vi "Remove User from Group.vi"(5 "Save File":bool=TRUE, 6 "error in (no error)":errorcluster, 7 "Group Name":string, 8 "LoginName":string, 9 "EasyUserManager in":refnum<class "EasyUserManager.lvclass">) -> (0 "error out":errorcluster, 3 "EasyUserManager out":refnum<class "EasyUserManager.lvclass">)   [LabVIEW 2024, in "EasyUserManager.lvclass"]
doc: "Remove the user specified by <B>LoginName</B> from the group specified by <B>Group Name</B>.\n\nThis VI will not do anything if the user is not a member of the group. \n\nThe boolean input <B>Save File</B> controls whether changes are immediately saved to the users file (Default: True)."
uses:
  EasyUserManager.lvclass
  EasyUserManager.lvclass/EasyUserManager.ctl
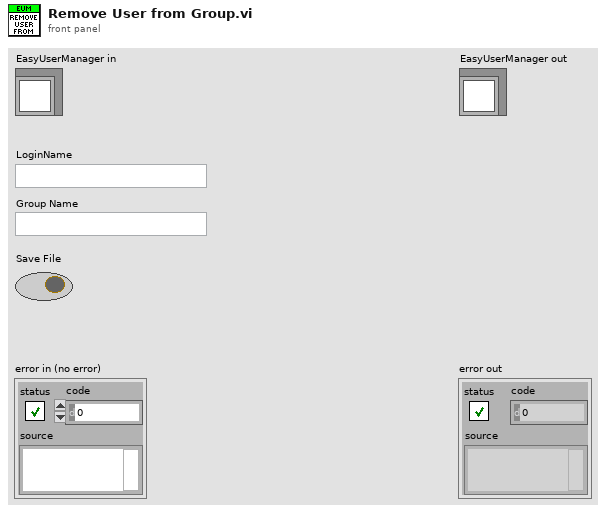
[diagram p1: front panel]
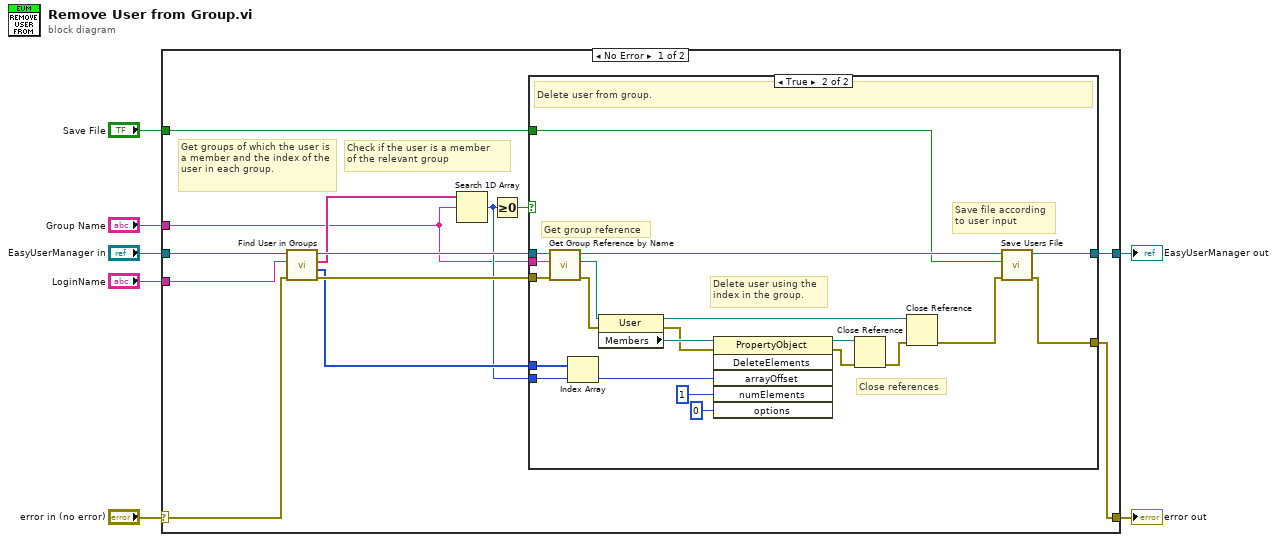
[diagram p0: block diagram]
diagram:
  n1 = case shown="No Error" "error in (no error)" {
    selector: "error in (no error)" -> [w11 w45]
    tunnel: [w19 w45] -> w6
    tunnel: [w20 w44] -> w4
    tunnel: "EasyUserManager in" -> [w17 w44]
    tunnel: "Save File" -> [w10 _]
    tunnel: "LoginName" -> [w9 _]
    tunnel: "Group Name" -> [w8 _]
    frame No Error {
      # "Check if the user is a member\nof the relevant group"
      # "Get groups of which the user is a member and the index of the user in each group."
      n2 = call "Find User in Groups.vi"("error in (no error)"=w11, "LoginName"=w9, "EasyUserManager in"=w17) -> ("error out"=w16:errorcluster, "Indexes"=w13:i32[], "Groups"=w15:string[], "EasyUserManager out"=w18:refnum<class "EasyUserManager.lvclass">)  [unwired: 1 in]
      n3 = Search 1D Array(1D array=w15, element=w8) -> (index of element=w12:i32)  [unwired: 1 in]
      n4 = Greater Or Equal To 0?(x=w12) -> (x >= 0?=w14:bool)
      n5 = case shown="True" w14 {
        tunnel: [w22 w43] -> w20
        tunnel: [w21 w42] -> w19
        tunnel: w18 -> [w22 w30]
        tunnel: w16 -> [w21 w29]
        tunnel: w8 -> [_ w27]
        tunnel: w13 -> [_ w26]
        tunnel: w12 -> [_ w25]
        tunnel: w10 -> [_ w23]
        frame False {
          # "User is not a member of the group. Do nothing."
        }
        frame True {
          # "Delete user using the \nindex in the group."
          # "Get group reference"
          # "Close references"
          # "Save file according\nto user input"
          # "Delete user from group."
          n6 = call "Get Group Reference by Name.vi"("error in (no error)"=w29, "Group Name"=w27, "EasyUserManager in"=w30) -> ("error out"=w32:errorcluster, "Group Reference"=w33:refnum<k7>, "EasyUserManager out"=w41:refnum<class "EasyUserManager.lvclass">)  [unwired: 2 in]
          n7 = Index Array(array=w26, index=w25) -> (element=w24:i32)
          n8 = property on="Property Node" class="User"(reference=w33, error in=w32) -> (reference out=w34:refnum<k7>, error out=w39:errorcluster, "Members"=w40:refnum<k7>)
          n9 = invoke on="Invoke Node" class="PropertyObject" method="DeleteElements"(reference=w40, error in=w39, "arrayOffset"=w24, "numElements"=1 ("options"), "options"=0 ("arrayOffset")) -> (reference out=w37:refnum<k7>, error out=w36:errorcluster)  [unwired: 1 in, 4 out]
          n10 = Close Reference(reference=w37, error in (no error)=w36) -> (error out=w35:errorcluster)
          n11 = Close Reference(reference=w34, error in (no error)=w35) -> (error out=w31:errorcluster)
          n12 = call "Save Users File.vi"("error in (no error)"=w31, "Save"=w23, "EasyUserManager in"=w41) -> ("error out"=w42:errorcluster, "EasyUserManager out"=w43:refnum<class "EasyUserManager.lvclass">)  [unwired: 3 in]
        }
      }
    }
    frame Error {
      # "Pass error and do nothing."
    }
  }
  "error out" <- w6
  "EasyUserManager out" <- w4
